vi "FuncVI-ss2str.vi"(5 "InstanceRef":T2, 9 "arg list":T1[](array[typedef]) {"num" format="%.2f"}) -> (0 "error out":bool, 3 "result":T1 {"num" format="%.2f"})   [LabVIEW 2021]
doc: "::: CalcExpress Toolkit :::\nCopyright (c) 2000-2026 Konstantin Shifershteyn. All rights reserved."
uses:
  cetypes.llb/CalcExpress Function Argument Info.ctl
  cetypes.llb/CalcExpress Instance RefNum.ctl
panel:
  in  "max arg num":i32=4
  in  "min arg num":i32=1
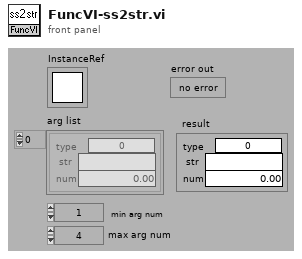
[diagram p1: front panel]
types:
  T1 = typedef "CalcExpress Function Argument Info.ctl" = cluster{"type":u32, "str":string, "num":dbl}
  T2 = typedef "CalcExpress Instance RefNum.ctl" = refnum<k1>
  T3 = cluster{"index":i32, "data type":enum32{"String", "DBL Number", "identifier", "1D Array of DBL", "2D Array of DBL", "CDB Number", "1D Array of CDB", "2D Array of CDB", "1D Array of String", "2D Array of String", "Unknown data type"}, "default num":dbl, "default str":string}[]
  T4 = cluster{"data type":enum32{"String", "DBL Number", "identifier", "1D Array of DBL", "2D Array of DBL", "CDB Number", "1D Array of CDB", "2D Array of CDB", "1D Array of String", "2D Array of String", "Unknown data type"}, "str":string, "num":dbl}
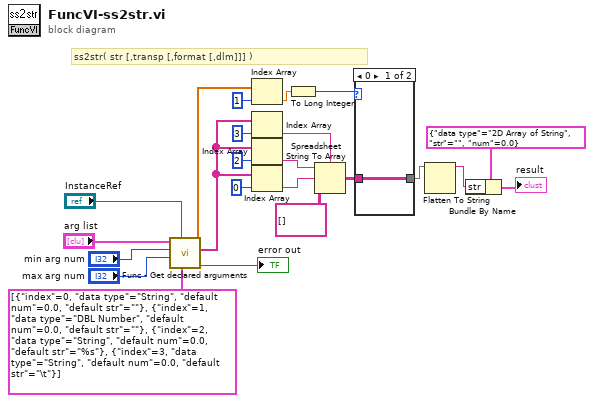
[diagram p0: block diagram]
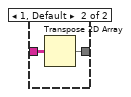
[diagram p2: hidden frame]
diagram:
  # "ss2str( str [,transp [,format [,dlm]]] )"
  n1 = call "Func - Get declared arguments.vi"("arg descriptors"=T3 [{"index"=0, "data type"=enum."String", "default num"=0.0, "default str"=""}, {"index"=1, "data type"=enum."DBL Number", "default num"=0.0, "default str"=""}, {"index"=2, "data type"=enum."String", "default num"=0.0, "default str"="%s"}, {"index"=3, "data type"=enum."String", "default num"=0.0, "default str"="\t"}] ("args descriptors"), "InstanceRef"="InstanceRef", "max arg num"="max arg num", "min arg num"="min arg num", "arg list"="arg list") -> ("error out"=→"error out":bool, "str list"=w13:string[], "num list"=w7:dbl[])  [unwired: 3 in, 1 out]
  n2 = Index Array(array=w7, index=1) -> (element=w6:dbl)
  n3 = Index Array(array=w13, index=3) -> (element=w18:string)
  n4 = Index Array(array=w13, index=2) -> (element=w19:string)
  n5 = Index Array(array=w13, index=0) -> (element=w12:string)
  n6 = To Long Integer(number=w6) -> (32bit integer=w5:i32)
  n7 = Spreadsheet String To Array(delimiter (Tab)=w18, format string=w19, spreadsheet string=w12, array type (2D Dbl)=string[][] []) -> (array=w4:string[][])
  n8 = case shown="0" w5 {
    tunnel: w4 -> [w24 w26]
    tunnel: [w24 w25] -> w3
    frame 0 {
    }
    frame 1, Default {
      n9 = Transpose 2D Array(2D array=w26) -> (transposed array=w25:string[][])
    }
  }
  n10 = Flatten To String(anything=w3) -> (data string=w9:string)  [unwired: 3 in, 2 out]
  n11 = Bundle By Name(cluster=T4 {"data type"=enum."2D Array of String", "str"="", "num"=0.0} ("opd info"), "str"=w9) -> (→"result":T4)
